vi "Hex2Bits.vi"(4 "Value":string) -> (1 "Bits":bool[](array[boolean]))   [LabVIEW 2025]
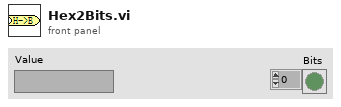
[diagram p1: front panel]
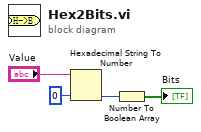
[diagram p0: block diagram]
diagram:
  n1 = Hexadecimal String To Number(string="Value", default (0uL)=u16 0 ("默认(0 U32)")) -> (number=w3:u16)  [unwired: 1 in, 1 out]
  n2 = Number To Boolean Array(number=w3) -> (Boolean array=→"Bits":bool[])
